vi "Set Channels.vi"(0 "record":cluster{"id":string, "Channels":set{i32}}, 5 "channel":i32, 11 "error in":errorcluster) -> (4 "record out":cluster{"id":string, "Channels":set{i32}}, 6 "channels":set{i32}(c389), 8 "already included?":bool, 15 "error out":errorcluster)   [LabVIEW 2026]
doc: "Adds a channel to a record's set of channels and reports whether it was new."
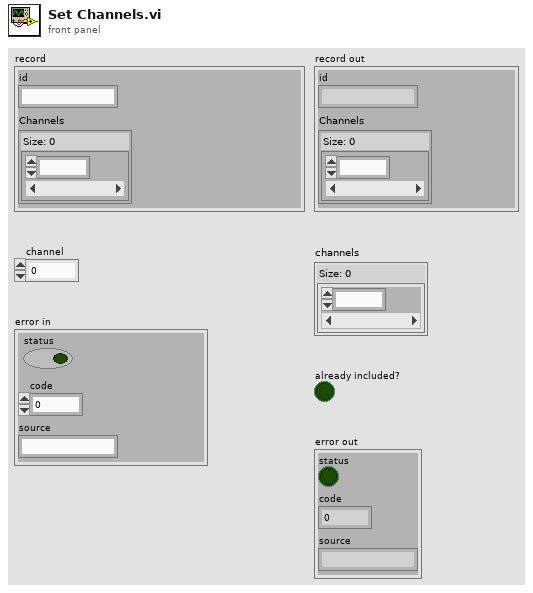
[diagram p1: front panel]
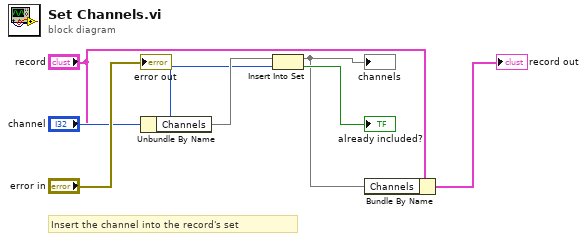
[diagram p0: block diagram]
diagram:
  # "Insert the channel into the record's set"
  n1 = Unbundle By Name("record") -> ("Channels"=w4:set{i32})
  n2 = Insert Into Set(10:"channel", 11:w4) -> (2:→"already included?":bool, 3:w5:set{i32})
  "channels" <- w5
  n3 = Bundle By Name(cluster="record", "Channels"=w5) -> (→"record out":cluster{"id":string, "Channels":set{i32}})
  "error out" <- "error in"
